vi "Test Suite.vi"   [LabVIEW 2026, in "Unit Tests.lvlib"]
uses:
  Unit Tests.lvlib
  <vilib>/addons/_JKI Toolkits/Caraya/classes/Test Suite/Define Test Suite (Default).vi
  <vilib>/addons/_JKI Toolkits/Caraya/classes/Test Suite/Test Suite.lvclass
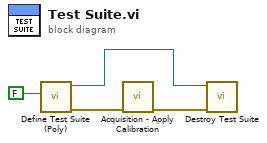
[diagram p0: block diagram]
diagram:
  n1 = call-poly <vilib>:"Define Test Suite (Poly).vi"("Interactive"=FALSE) -> ("error out"=w4:errorcluster, "Test Suite"=w2:refnum<class "Test Suite.lvclass">)  [unwired: 8 in, 1 out]
  n2 = call "Acquisition - Apply Calibration.vi"("error in (no error)"=w4) -> ("error out"=w1:errorcluster)  [unwired: 10 in]
  n3 = call-dynamic "Destroy Test Suite.vi"("error in (no error)"=w1, "Test Suite in"=w2) -> ()  [unwired: 8 in, 2 out]
